vi "Create Message VI (from Accessor).vi"(8 "error in (no error)":errorcluster, 9 "accessor type":T1="Get", 10 "rpc message name":string, 11 "rpc messages folder in":refnum<vi>) -> (0 "error out":errorcluster, 1 "created?":bool, 2 "accessor vi":refnum<vi>, 3 "rpc messages folder out":refnum<vi>)   [LabVIEW 2019, in "gRPC Template Creation Utility.lvlib"]
uses:
  gRPC Template Creation Utility.lvlib
  TypeDefs/Method Accessor Type.ctl
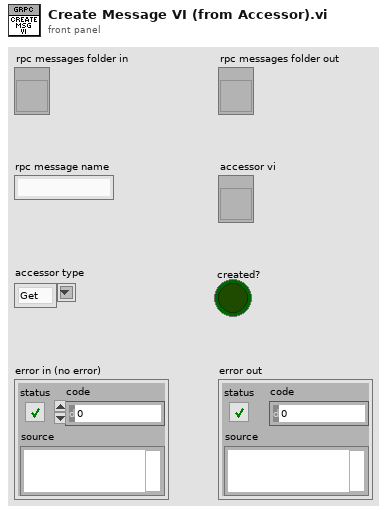
[diagram p1: front panel]
types:
  T1 = typedef "gRPC Template Creation Utility.lvlib/Method Accessor Type.ctl" = string
  T2 = enum32{"invalid VI type", "Standard VI", "Control VI", "Global VI", "Polymorphic VI", "Configuration VI", "SubSystem", "Facade VI", "Method VI"}
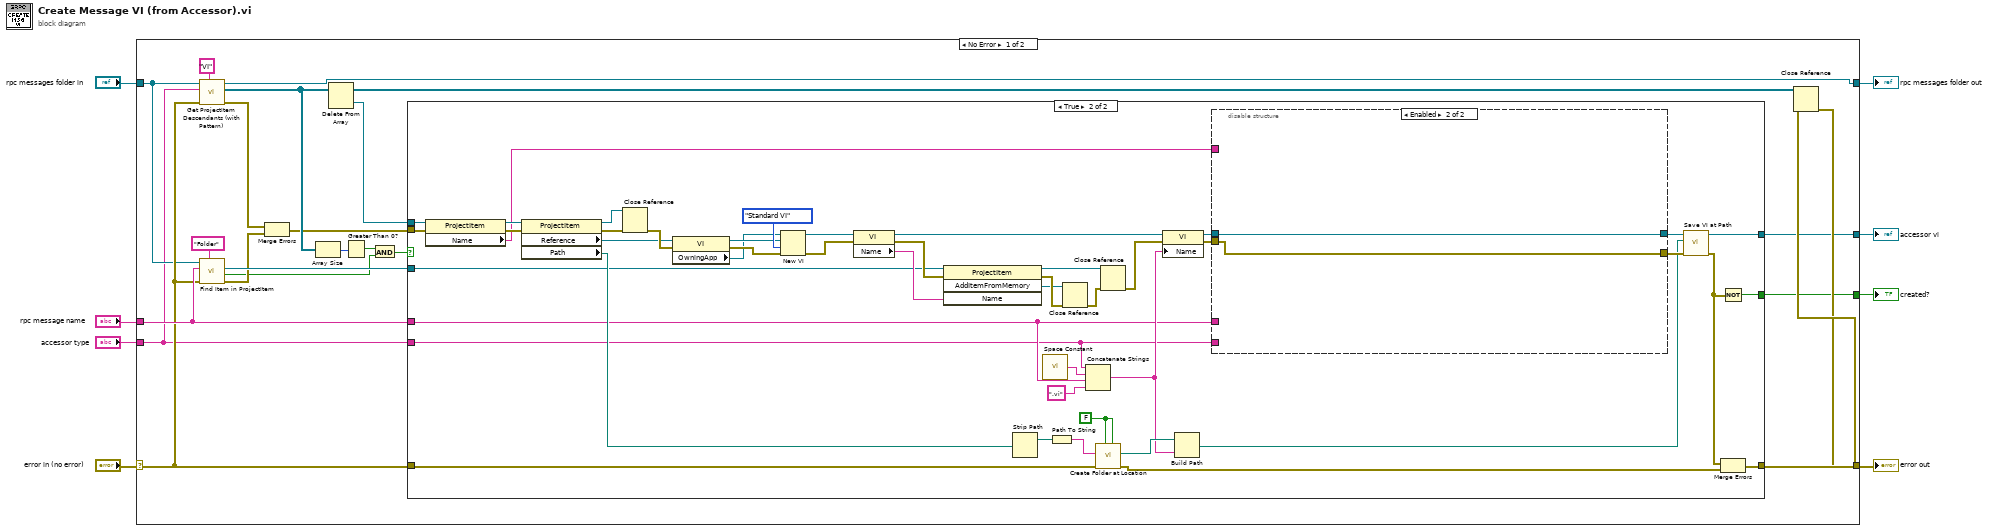
[diagram p0: block diagram]
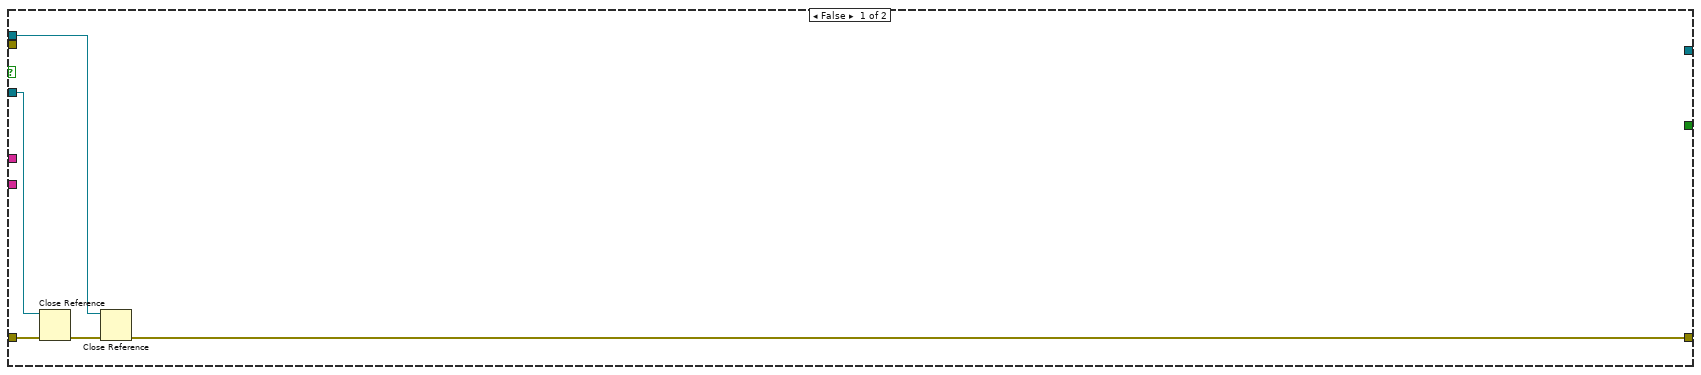
[diagram p2: hidden frame]
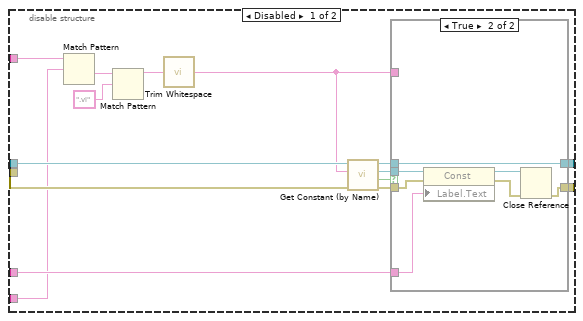
[diagram p3: hidden frame]
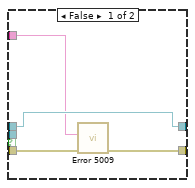
[diagram p4: hidden frame]
diagram:
  n1 = case shown="No Error" "error in (no error)" {
    selector: "error in (no error)" -> [w16 w110]
    tunnel: "rpc message name" -> [w26 _]
    tunnel: "rpc messages folder in" -> [w10 w109]
    tunnel: [w14 w110] -> w5
    tunnel: [w13 w109] -> w4
    tunnel: [w12 _] -> w3
    tunnel: [w11 _] -> w2
    tunnel: "accessor type" -> [w9 _]
    frame No Error {
      n2 = call "Get ProjectItem Descendants (with Pattern).vi"("Type"="VI", "error in (no error)"=w16, "Pattern"=w9, "ProjectItem in"=w10) -> ("error out"=w20:errorcluster, "ProjectItem descendents"=w25:refnum<vi>[], "ProjectItem out"=w13:refnum<vi>)  [unwired: 5 in]
      n3 = call "Find Item in ProjectItem.vi"("Item Type"="Folder", "error in (no error)"=w16, "Name"=w26, "ProjectItem in"=w10) -> ("error out"=w19:errorcluster, "Found ?"=w18:bool, "Item Refnum out"=w23:refnum<vi>)  [unwired: 4 in, 1 out]
      n4 = Merge Errors(w20, w19) -> (w17:errorcluster)
      n5 = Array Size(array=w25) -> (size(s)=w24:i32)
      n6 = Delete From Array(array=w25) -> (deleted portion=w28:refnum<vi>, array with subset deleted=w30:refnum<vi>[])  [unwired: 2 in]
      n7 = Greater Than 0?(x=w24) -> (x > 0?=w22:bool)
      n8 = And(x=w22, y=w18) -> (x .and. y?=w21:bool)
      n9 = case shown="True" w21 {
        tunnel: w26 -> [_ w42]
        tunnel: [w31 w78] -> w15
        tunnel: [_ w48] -> w11
        tunnel: w28 -> [w35 w55]
        tunnel: [_ w64] -> w12
        tunnel: w23 -> [w34 w60]
        tunnel: w16 -> [w33 w59]
        tunnel: w17 -> [_ w54]
        tunnel: w9 -> [_ w41]
        frame False {
          n10 = Close Reference(reference=w34, error in (no error)=w33) -> (error out=w32:errorcluster)
          n11 = Close Reference(reference=w35, error in (no error)=w32) -> (error out=w31:errorcluster)
        }
        frame True {
          w76 = FALSE ("Use Relative (F)")
          n12 = property class="ProjectItem"(reference=w55, error in=w54) -> (reference out=w53:refnum<vi>, error out=w52:errorcluster, "Name"=w43:string)
          n13 = property class="ProjectItem"(reference=w53, error in=w52) -> (reference out=w80:refnum<vi>, error out=w79:errorcluster, "Reference"=w38:refnum<vi>, "Path"=w72:path)
          n14 = Close Reference(reference=w80, error in (no error)=w79) -> (error out=w40:errorcluster)
          n15 = property class="VI"(reference=w38, error in=w40) -> (reference out=w37:refnum<vi>, error out=w39:errorcluster, "OwningApp"=w36:refnum<vi>)
          n16 = New VI(8:w39, 9:T2."Standard VI" ("vi type (standard vi)"), 10:w37, 11:w36) -> (0:w69:errorcluster, 3:w67:refnum<vi>)  [unwired: 3 out]
          n17 = property class="VI"(reference=w67, error in=w69) -> (reference out=w73:refnum<vi>, error out=w74:errorcluster, "Name"=w70:string)
          n18 = invoke class="ProjectItem" method="AddItemFromMemory"(reference=w60, error in=w74, "Name"=w70) -> (reference out=w66:refnum<vi>, error out=w58:errorcluster, "AddItemFromMemory"=w57:refnum<vi>)  [unwired: 1 in, 1 out]
          n19 = Strip Path(path=w72) -> (stripped path=w44:path)  [unwired: 1 out]
          n20 = call <vilib>:"Space Constant.vi"() -> ("String"=w63:string)
          n21 = Path To String(path=w44) -> (string=w71:string)
          n22 = Close Reference(reference=w57, error in (no error)=w58) -> (error out=w56:errorcluster)
          n23 = Concatenate Strings(w41, w63, w42, ".vi" ("string")) -> (w61:string)
          n24 = call "Create Folder at Location.vi"("Override existing (F)"=w76, "Use Relative (F)"=w76, "Error In"=w59, "Path"=w71) -> ("Error Out"=w77:errorcluster, "Full path out"=w75:path)  [unwired: 5 in, 1 out]
          n25 = Close Reference(reference=w66, error in (no error)=w56) -> (error out=w65:errorcluster)
          n26 = property class="VI"(reference=w73, error in=w65, "Name"=w61) -> (reference out=w51:refnum<vi>, error out=w50:errorcluster)
          n27 = Build Path(base path=w75, name or relative path=w61) -> (appended path=w47:path)
          n28 = disable-structure shown="Enabled" {
            disable-tunnel: w51 -> [w94 w108]
            disable-tunnel: w50 -> [w93 w107]
            disable-tunnel: w42 -> [w92 _]
            disable-tunnel: [w90 w107] -> w49
            disable-tunnel: [w87 w108] -> w45
            disable-tunnel: w43 -> [w83 _]
            disable-tunnel: w41 -> [w81 _]
            frame Disabled {
              n29 = Match Pattern(string=w83, regular expression=w81) -> (after substring=w85:string)  [unwired: 1 in, 3 out]
              n30 = Match Pattern(string=w85, regular expression=".vi") -> (before substring=w86:string)  [unwired: 1 in, 3 out]
              n31 = call <vilib>:"Trim Whitespace.vi"("string"=w86) -> ("trimmed string"=w82:string)  [unwired: 1 in]
              n32 = call "Get Constant (by Name).vi"("error in (no error)"=w93, "Constant Label"=w82, "Owner VI in"=w94) -> ("error out"=w91:errorcluster, "Found ?"=w89:bool, "Const ref out"=w95:refnum<vi>, "Owner VI out"=w88:refnum<vi>)  [unwired: 5 in]
              n33 = case shown="True" w89 {
                tunnel: w95 -> [_ w106]
                tunnel: w92 -> [_ w105]
                tunnel: w91 -> [w98 w104]
                tunnel: [w97 w101] -> w90
                tunnel: w88 -> [w99 w100]
                tunnel: [w99 w100] -> w87
                tunnel: w82 -> [w96 _]
                frame False {
                  n34 = call "Error 5009.vi"("error in (no error)"=w98, "Cluster Definition Constant"=w96) -> ("error out"=w97:errorcluster)  [unwired: 9 in]
                }
                frame True {
                  n35 = property class="Const"(reference=w106, error in=w104, "Label.Text"=w105) -> (reference out=w103:refnum<vi>, error out=w102:errorcluster)
                  n36 = Close Reference(reference=w103, error in (no error)=w102) -> (error out=w101:errorcluster)
                }
              }
            }
            frame Enabled {
            }
          }
          n37 = call "Save VI at Path.vi"("error in (no error)"=w49, "Path"=w47, "VI in"=w45) -> ("error out"=w46:errorcluster, "VI out"=w48:refnum<vi>)  [unwired: 6 in, 1 out]
          n38 = Not(x=w46) -> (.not. x?=w64:bool)
          n39 = Merge Errors(w46, w77) -> (w78:errorcluster)
        }
      }
      n40 = Close Reference(reference=w30, error in (no error)=w15) -> (error out=w14:errorcluster)
    }
    frame Error {
    }
  }
  "error out" <- w5
  "rpc messages folder out" <- w4
  "created?" <- w3
  "accessor vi" <- w2
